vi "ProgramControlAccess.vi"(0 "Program Interface in":refnum<class "Program Interface.lvclass">, 1 "Program Status":T1, 5 "error in (no error)":errorcluster, 8 "Robot Status":T3) -> (14 "Program Interface out":refnum<class "Program Interface.lvclass">, 19 "error out":errorcluster)   [LabVIEW 2019, in "Program Interface.lvclass"]
uses:
  Program Interface.lvclass
  Robot/Universal Robot/RobotStatus.ctl
  Robot/Universal Robot/RobotMode.ctl
  Robot/Universal Robot/OperationalMode.ctl
  Robot/Universal Robot/SafetyStatus.ctl
  Robot/Universal Robot/ProgramStatus.ctl
  Robot/Universal Robot/ProgramState.ctl
  Program Interface.lvclass/Program Interface.ctl
  Robot/Universal Robot/Universal Robot.lvclass
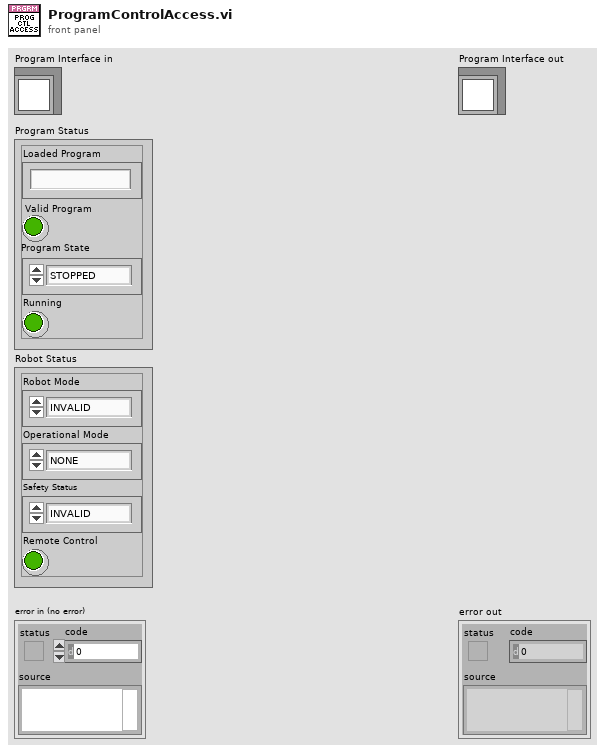
[diagram p1: front panel]
types:
  T1 = typedef "Universal Robot.lvclass/ProgramStatus.ctl" = cluster{"Loaded Program":string, "Valid Program":bool, "Program State":T2, "Running":bool}
  T2 = typedef "Universal Robot.lvclass/ProgramState.ctl" = enum16{"STOPPED", "PLAYING", "PAUSE"}
  T3 = typedef "Universal Robot.lvclass/RobotStatus.ctl" = cluster{"Robot Mode":T4, "Operational Mode":T5, "Safety Status":T6, "Remote Control":bool}
  T4 = typedef "Universal Robot.lvclass/RobotMode.ctl" = enum16{"INVALID", "NO_CONTROLLER", "DISCONNECTED", "CONFIRM_SAFETY", "BOOTING", "POWER_OFF", "POWER_ON", "IDLE", "BACKDRIVE", "RUNNING"}
  T5 = typedef "Universal Robot.lvclass/OperationalMode.ctl" = enum16{"NONE", "MANUAL", "AUTOMATIC"}
  T6 = typedef "Universal Robot.lvclass/SafetyStatus.ctl" = enum16{"INVALID", "NORMAL", "REDUCED", "PROTECTIVE_STOP", "RECOVERY", "SAFEGUARD_STOP", "SYSTEM_EMERGENCY_STOP", "ROBOT_EMERGENCY_STOP", "VIOLATION", "FAULT", "AUTOMATIC_MODE_SAFEGAURD_STOP", "SYSTEM_THREE_POSITION_ENABLING_STOP"}
  T7 = enum8{"Enabled", "Disabled", "Disabled and Grayed Out"}
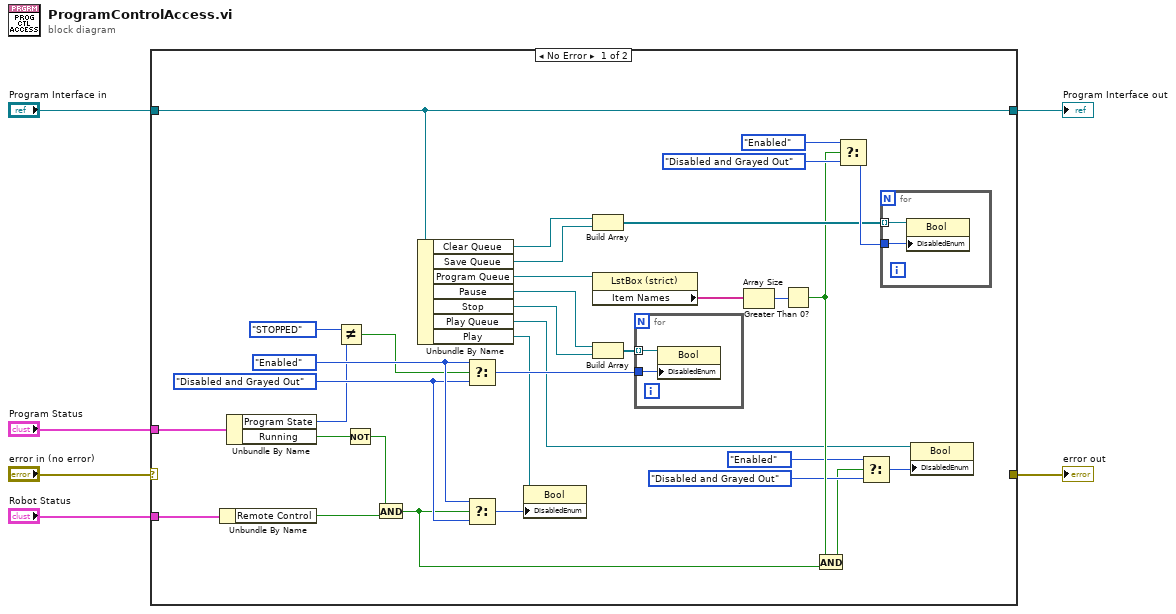
[diagram p0: block diagram]
diagram:
  n1 = case shown="No Error" "error in (no error)" {
    selector: "error in (no error)" -> [_ w45]
    tunnel: [_ w45] -> w5
    tunnel: [w39 w44] -> w3
    tunnel: "Program Interface in" -> [w39 w44]
    tunnel: "Robot Status" -> [w38 _]
    tunnel: "Program Status" -> [w35 _]
    frame No Error {
      w33 = T7."Disabled and Grayed Out" ("Disabled")
      w34 = T7."Enabled" ("Disabled")
      n2 = Unbundle By Name(w38) -> ("Remote Control"=w7:bool)
      n3 = Unbundle By Name(w35) -> ("Program State"=w20:T2, "Running"=w31:bool)
      n4 = Not Equal?(x=ProgramState."STOPPED", y=w20) -> (x != y?=w18:bool)
      n5 = Not(x=w31) -> (.not. x?=w30:bool)
      n6 = And(x=w30, y=w7) -> (x .and. y?=w12:bool)
      n7 = Unbundle By Name(w39) -> ("Clear Queue"=w23:refnum<vi>, "Save Queue"=w22:refnum<vi>, "Program Queue"=w29:refnum<vi>, "Pause"=w36:refnum<vi>, "Stop"=w37:refnum<vi>, "Play Queue"=w13:refnum<vi>, "Play"=w14:refnum<vi>)
      n8 = Select(t=w34, s=w18, f=w33) -> (s? t:f=w16:T7)
      n9 = Select(t=w34, s=w12, f=w33) -> (s? t:f=w32:T7)
      n10 = property class="Bool"(reference=w14, "DisabledEnum"=w32) -> ()  [unwired: 1 in, 2 out]
      n11 = Build Array(w23, w22) -> (w21:refnum<vi>[])
      n12 = property class="LstBox (strict)"(reference=w29) -> ("Item Names"=w28:string[])  [unwired: 1 in, 2 out]
      n13 = Build Array(w36, w37) -> (w17:refnum<vi>[])
      n14 = for {
        tunnel: w17 -> [w41] mode=indexing
        tunnel: w16 -> [w40]
        n15 = property class="Bool"(reference=w41, "DisabledEnum"=w40) -> ()  [unwired: 1 in, 2 out]
      }
      n16 = Array Size(array=w28) -> (size(s)=w27:i32)
      n17 = Greater Than 0?(x=w27) -> (x > 0?=w15:bool)
      n18 = And(x=w15, y=w12) -> (x .and. y?=w8:bool)
      n19 = Select(t=T7."Enabled" ("Disabled"), s=w15, f=T7."Disabled and Grayed Out" ("Disabled")) -> (s? t:f=w24:T7)
      n20 = Select(t=T7."Enabled" ("Disabled"), s=w8, f=T7."Disabled and Grayed Out" ("Disabled")) -> (s? t:f=w9:T7)
      n21 = for {
        tunnel: w24 -> [w43]
        tunnel: w21 -> [w42] mode=indexing
        n22 = property class="Bool"(reference=w42, "DisabledEnum"=w43) -> ()  [unwired: 1 in, 2 out]
      }
      n23 = property class="Bool"(reference=w13, "DisabledEnum"=w9) -> ()  [unwired: 1 in, 2 out]
    }
    frame Error {
    }
  }
  "error out" <- w5
  "Program Interface out" <- w3
